vi "New VI Swap Probe NI.vi"(0 "password":string, 11 "error in":errorcluster) -> (15 "error out":errorcluster)   [LabVIEW 2026]
doc: "Probe: New VI takes password as a string."
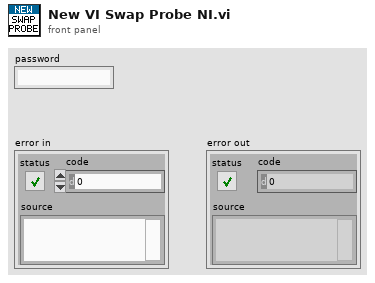
[diagram p1: front panel]
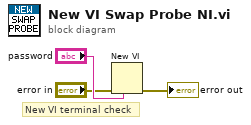
[diagram p0: block diagram]
diagram:
  # "New VI terminal check"
  n1 = New VI(6:"password", 8:"error in") -> (0:→"error out":errorcluster)  [unwired: 5 in, 1 out]
